vi "RDC-water-generate_all_perm.vi"(5 "Increment f (10MHz)":dbl=10000000.0, 7 "Stop f (6GHz) 2":dbl=6000000000.0, 8 "temp step [0.1C]":dbl=0.1, 9 "stop temp [10-40C]":dbl=40.0, 10 "start temp [10-40C]":dbl=10.0, 11 "Start f (300MHz)":dbl=300000000.0) -> (0 "temp Array":dbl[](array[numeric]), 1 "complex":cluster{dbl[], cdb[]}[](array[cluster]), 2 "Real":cluster{dbl[], dbl[]}[](array[cluster]), 3 "Image":cluster{dbl[], dbl[]}[](array[cluster]))   [LabVIEW 2020, in "RDC-Reflection_Data_Computation.lvlib"]
doc: "Generates the water model permittivity for a range of temperatures (10-40 C) and frequencies. Returns the temperatures and the complex, real and imaginary permittivity per temperature; can save each set as a common-format file."
uses:
  RDC-Reflection_Data_Computation.lvlib
  Reflector/RFH-common_data_format.ctl
  Reflector/RFH-Reflection_File_Handler.lvlib
panel:
  in  "save":bool
  in  "Path":path=path "C:/projects/Universitet/Master/data/watertemp/convert water/water"
  out "imag":cluster{dbl[], dbl[]}[](graph)
  out "real":cluster{dbl[], dbl[]}[](graph)
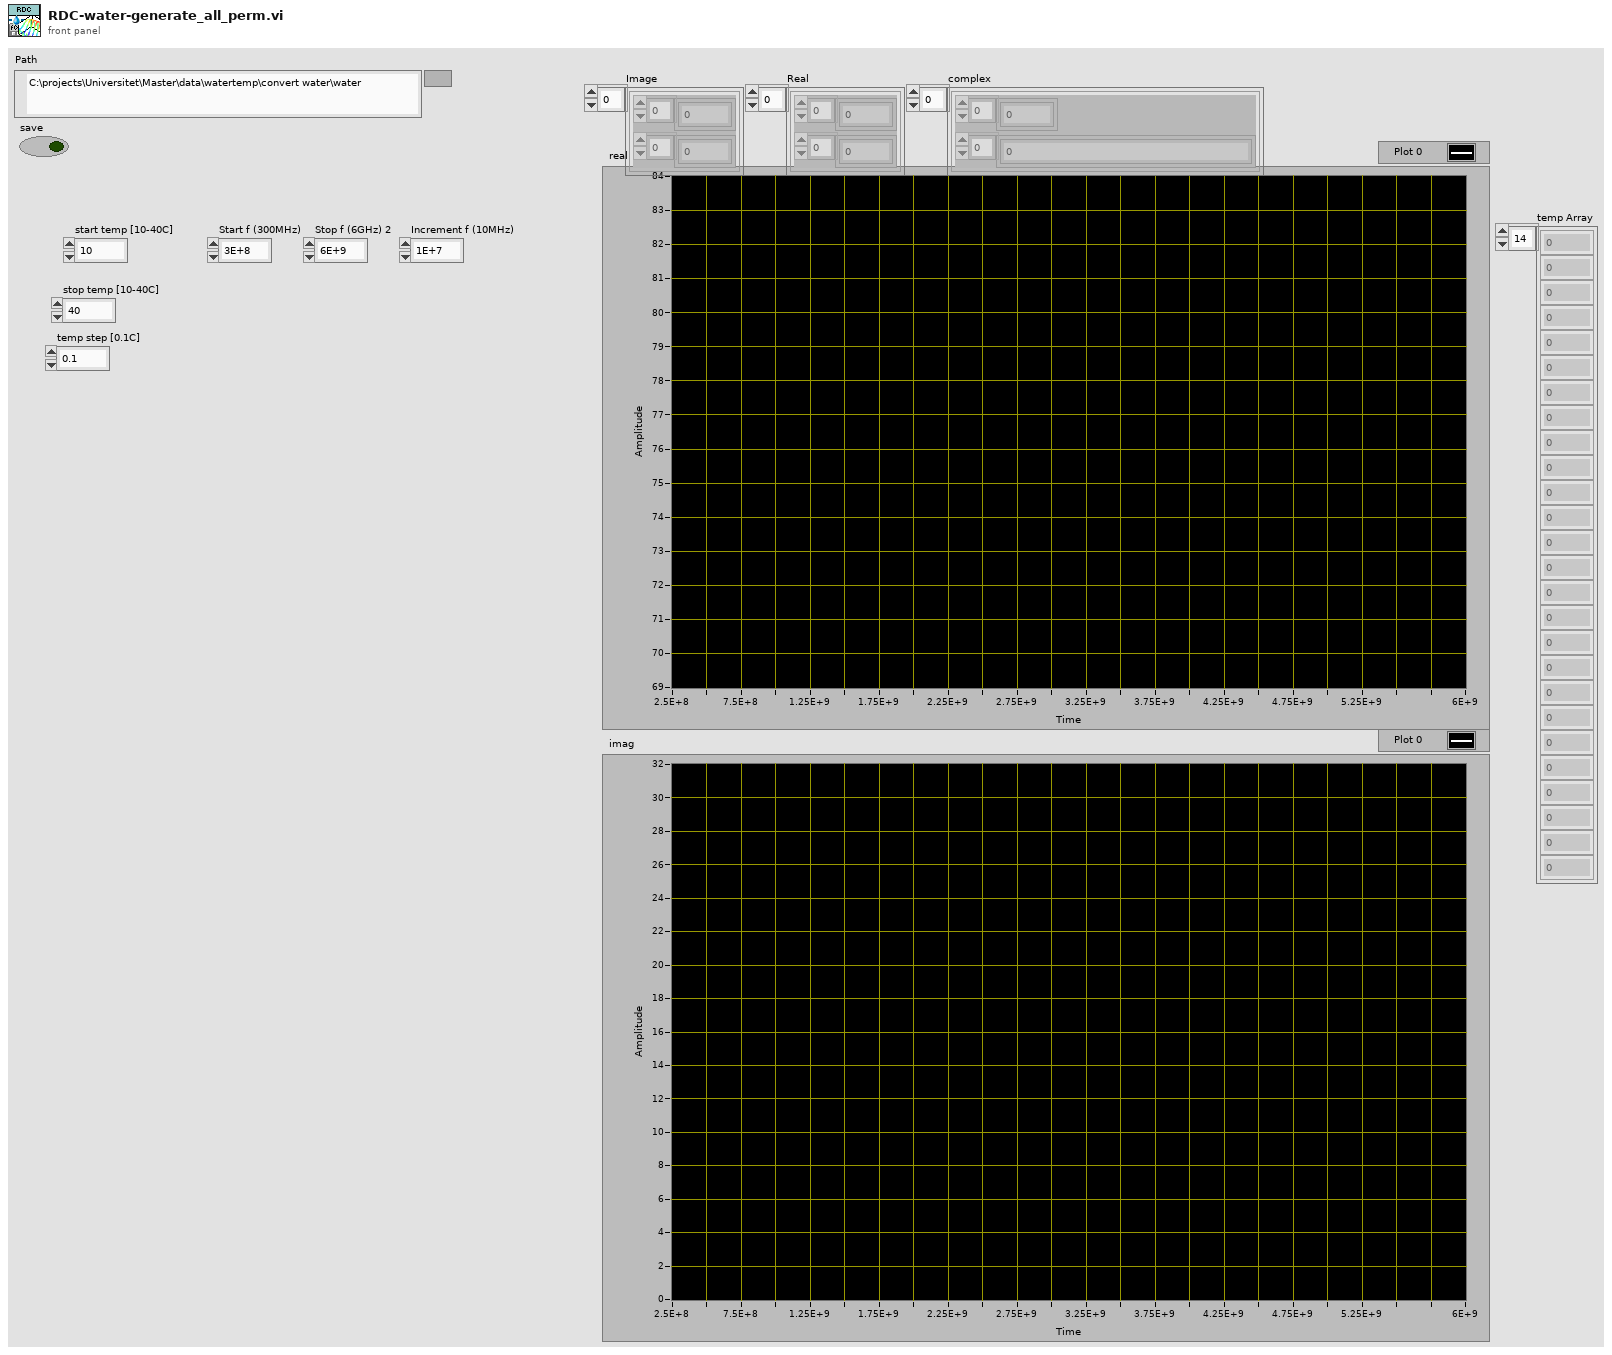
[diagram p1: front panel]
types:
  T1 = typedef "RFH-Reflection_File_Handler.lvlib/RFH-common_data_format.ctl" = cluster{"Frequency":dbl[], "Reflection'":dbl[], "Reflection''":dbl[], "Permativity'":dbl[], "Permativity''":dbl[], "Conductivity":dbl[], "Loss Tangent":dbl[], "Resistance":dbl[], "Reactance":dbl[]}
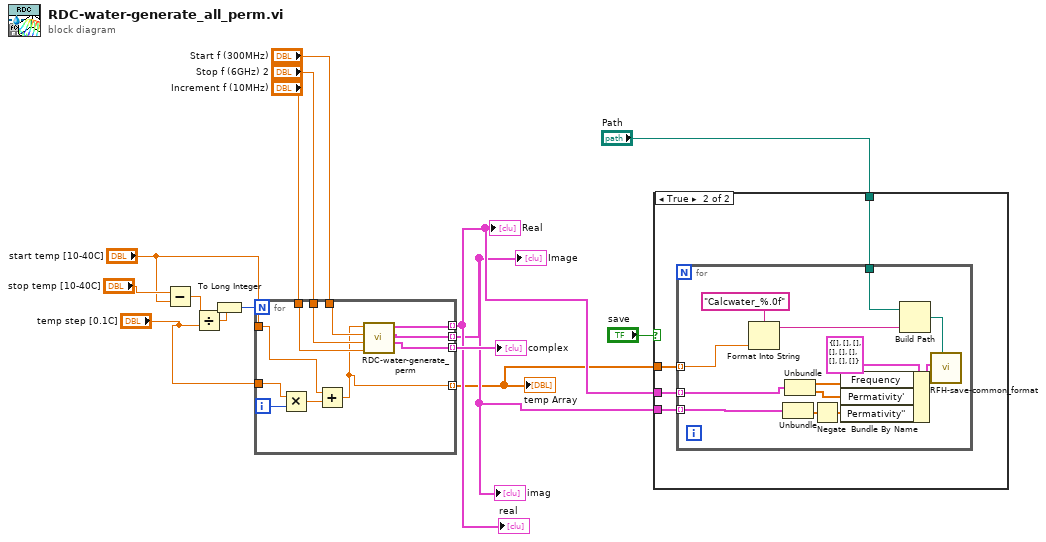
[diagram p0: block diagram]
diagram:
  n1 = Subtract(x="stop temp [10-40C]", y="start temp [10-40C]") -> (x-y=w10:dbl)
  n2 = Divide(x=w10, y="temp step [0.1C]") -> (x/y=w8:dbl)
  n3 = To Long Integer(number=w8) -> (32bit integer=w7:i32)
  n4 = for {
    N: w7 -> [_]
    tunnel: "start temp [10-40C]" -> [w20]
    tunnel: "Start f (300MHz)" -> [w26]
    tunnel: "Stop f (6GHz) 2" -> [w25]
    tunnel: "Increment f (10MHz)" -> [w24]
    tunnel: "temp step [0.1C]" -> [w22]
    tunnel: [w19] -> w3 mode=indexing
    tunnel: [w18] -> w5 mode=indexing
    tunnel: [w17] -> w4 mode=indexing
    tunnel: [w16] -> w6 mode=indexing
    i -> [w23]
    n5 = Multiply(x=w22, y=w23) -> (x*y=w21:dbl)
    n6 = Add(x=w20, y=w21) -> (x+y=w19:dbl)
    n7 = call "RDC-water-generate_perm.vi"("Increment f (10MHz)"=w24, "Stop f (6GHz) 2"=w25, "Start f (300MHz)"=w26, "water Temp (25C) [10-40C]"=w19) -> ("Complex Perm"=w16:cluster{dbl[], cdb[]}, "Imag Perm"=w17:cluster{dbl[], dbl[]}, "Real Perm"=w18:cluster{dbl[], dbl[]})  [unwired: 3 in, 2 out]
  }
  "temp Array" <- w3
  "imag" <- w4
  "Image" <- w4
  "Real" <- w5
  "complex" <- w6
  "real" <- w5
  n8 = case shown="True" "save" {
    tunnel: w5 -> [_ w30]
    tunnel: w4 -> [_ w29]
    tunnel: w3 -> [_ w28]
    tunnel: "Path" -> [_ w27]
    frame False {
    }
    frame True {
      n9 = for {
        tunnel: w30 -> [w34] mode=indexing
        tunnel: w29 -> [w33] mode=indexing
        tunnel: w28 -> [w32] mode=indexing
        tunnel: w27 -> [w31]
        n10 = Format Into String(format string="Calcwater_%.0f", w32) -> (resulting string=w37:string)  [unwired: 2 in, 1 out]
        n11 = Unbundle(w33) -> (w39:dbl[])  [unwired: 1 out]
        n12 = Unbundle(w34) -> (w41:dbl[], w40:dbl[])
        n13 = Negate(x=w39) -> (-x=w35:dbl[])
        n14 = Bundle By Name(cluster=T1 {"Frequency"=[], "Reflection'"=[], "Reflection''"=[], "Permativity'"=[], "Permativity''"=[], "Conductivity"=[], "Loss Tangent"=[], "Resistance"=[], "Reactance"=[]} ("Common Format"), "Frequency"=w41, "Permativity'"=w40, "Permativity''"=w35) -> (w42:T1)
        n15 = Build Path(base path=w31, name or relative path=w37) -> (appended path=w36:path)
        n16 = call "RFH-save-common_format.vi"("file path (use dialog)"=w36, "Common Format"=w42) -> ()  [unwired: 9 in, 1 out]
      }
    }
  }
